vi "NR check RB Size.vi"(8 "error in (no error)":errorcluster caption="에러 입력(에러 없음)", 10 "RB Value (0~273)":i32, 11 "Instrument Manager 입력":refnum<class "Instrument Manager.lvclass">) -> (0 "error out":errorcluster caption="에러 출력", 2 "Success?":bool, 3 "Instrument Manager 출력":refnum<class "Instrument Manager.lvclass">)   [LabVIEW 2023, in "Instrument Manager.lvclass"]
uses:
  Instrument Manager.lvclass
  Instrument Manager.lvclass/Instrument Manager.ctl
  Module/ANRITSU Call Box/Type Definition/NR RB Setting Params for query.ctl
  Module/ANRITSU Call Box/ANRITSU Call Box.lvlib
  Module/ANRITSU Call Box/Interface Class/Anritsu Call Box.lvclass
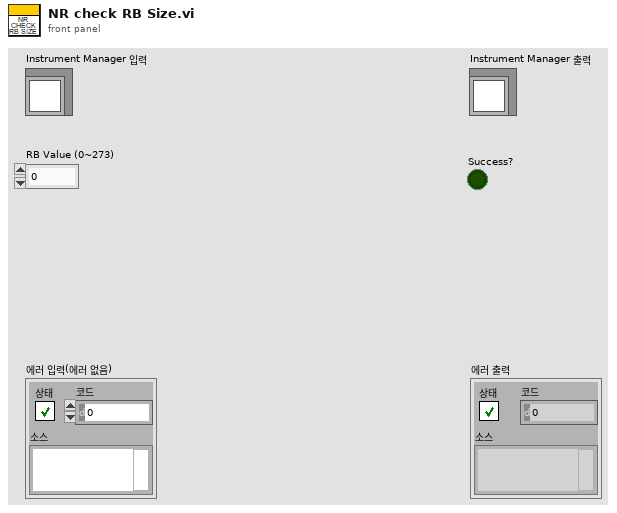
[diagram p1: front panel]
types:
  T1 = typedef "ANRITSU Call Box.lvlib/NR RB Setting Params for query.ctl" = cluster{"Selected CC":enum16{"PCC", "SCC", "FR2_PCC", "FR2_SCC"}, "RB Setting Type":enum16{"Number of RB", "Starting RB"}, "SCC or FR2_SCC Index":u32}
  T2 = cluster{"Anritsu Call Box":refnum<class "Anritsu Call Box.lvclass">, "Spectrum Analyzer":refnum<class "Interface_Spectrum.lvclass">, "RF Switch Box":refnum<class "RF Filter Box.lvclass">, "Turn Table":refnum<class "Interface - Turn Table.lvclass">, "Mast":refnum<class "Interface - Mast.lvclass">, "3D Controller":refnum<class "Interface_3D Controller.lvclass">}
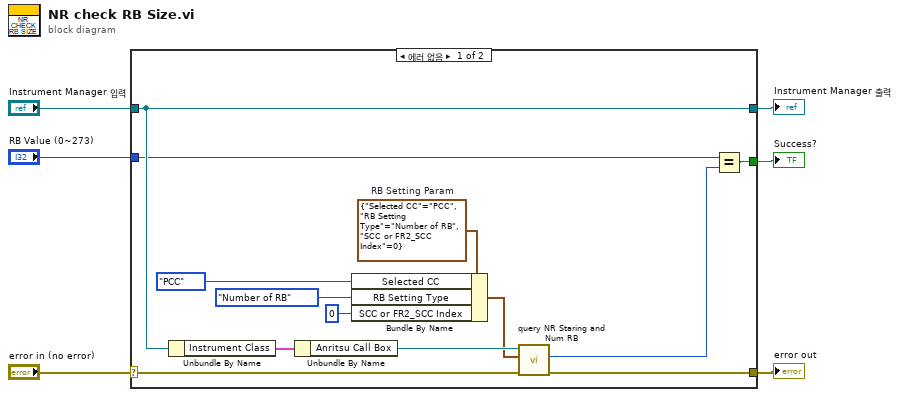
[diagram p0: block diagram]
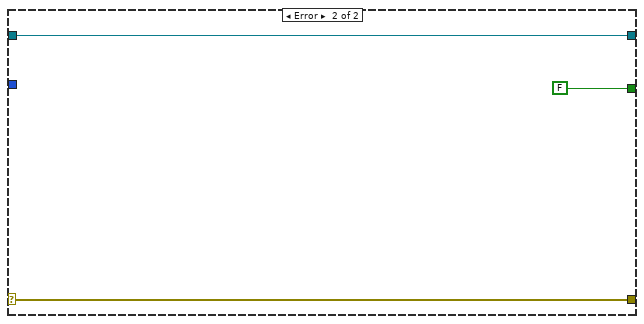
[diagram p2: hidden frame]
diagram:
  n1 = case shown="에러 없음" "error in (no error)" {
    selector: "error in (no error)" -> [w17 w22]
    tunnel: [w10 w22] -> w5
    tunnel: [w19 w21] -> w3
    tunnel: "Instrument Manager 입력" -> [w19 w21]
    tunnel: "RB Value (0~273)" -> [w8 _]
    tunnel: [w7 FALSE] -> w1
    frame No Error {
      w15 = T1 {"Selected CC"=enum."PCC", "RB Setting Type"=enum."Number of RB", "SCC or FR2_SCC Index"=0}  # RB Setting Param
      n2 = Unbundle By Name(w19) -> ("Instrument Class"=w18:T2)
      n3 = Unbundle By Name(w18) -> ("Anritsu Call Box"=w16:refnum<class "Anritsu Call Box.lvclass">)
      n4 = Bundle By Name(cluster=w15, "Selected CC"=enum16{"PCC", "SCC", "FR2_PCC", "FR2_SCC"}."PCC", "RB Setting Type"=enum16{"Number of RB", "Starting RB"}."Number of RB", "SCC or FR2_SCC Index"=u32 0) -> (w14:T1)
      n5 = call-dynamic "query NR Staring and Num RB.vi"("error in (no error)"=w17, "RB Setting Param"=w14, "Anritsu Call Box in"=w16) -> ("error out"=w10:errorcluster, "RB Value (0~273)"=w9:i32)  [unwired: 6 in, 1 out]
      n6 = Equal?(x=w8, y=w9) -> (x = y?=w7:bool)
    }
    frame Error {
    }
  }
  "error out" <- w5
  "Instrument Manager 출력" <- w3
  "Success?" <- w1
